vi "NR set HO Band.vi"(8 "error in (no error)":errorcluster caption="에러 입력(에러 없음)", 10 "Operation Band":u32, 11 "Instrument Manager 입력":refnum<class "Instrument Manager.lvclass">) -> (0 "error out":errorcluster caption="에러 출력", 3 "Instrument Manager 출력":refnum<class "Instrument Manager.lvclass">)   [LabVIEW 2023, in "Instrument Manager.lvclass"]
uses:
  Instrument Manager.lvclass
  Module/ANRITSU Call Box/Type Definition/NR Selected CC Type Arguments.ctl
  Instrument Manager.lvclass/Instrument Manager.ctl
  Module/ANRITSU Call Box/Interface Class/Anritsu Call Box.lvclass
  Module/ANRITSU Call Box/ANRITSU Call Box.lvlib
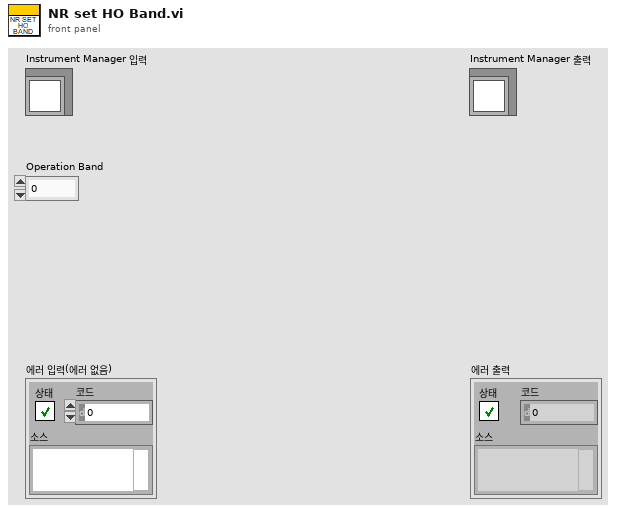
[diagram p1: front panel]
types:
  T1 = typedef "ANRITSU Call Box.lvlib/NR Selected CC Type Arguments.ctl" = cluster{"Selected CC":enum16{"PCC", "SCC", "FR2_PCC", "FR2_SCC"}, "SCC or FR2_SCC Index":u32}
  T2 = cluster{"Anritsu Call Box":refnum<class "Anritsu Call Box.lvclass">, "Spectrum Analyzer":refnum<class "Interface_Spectrum.lvclass">, "RF Switch Box":refnum<class "RF Filter Box.lvclass">, "Turn Table":refnum<class "Interface - Turn Table.lvclass">, "Mast":refnum<class "Interface - Mast.lvclass">, "3D Controller":refnum<class "Interface_3D Controller.lvclass">}
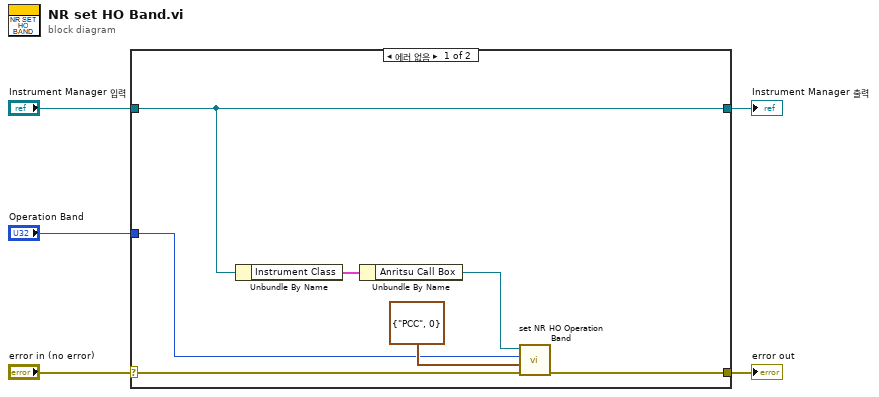
[diagram p0: block diagram]
diagram:
  n1 = case shown="에러 없음" "error in (no error)" {
    selector: "error in (no error)" -> [w11 w14]
    tunnel: [w10 w14] -> w4
    tunnel: [w8 w13] -> w2
    tunnel: "Instrument Manager 입력" -> [w8 w13]
    tunnel: "Operation Band" -> [w9 _]
    frame No Error {
      n2 = Unbundle By Name(w8) -> ("Instrument Class"=w7:T2)
      n3 = Unbundle By Name(w7) -> ("Anritsu Call Box"=w6:refnum<class "Anritsu Call Box.lvclass">)
      n4 = call-dynamic "set NR HO Operation Band.vi"("error in (no error)"=w11, "Selected CC Argements"=T1 {"Selected CC"=enum."PCC", "SCC or FR2_SCC Index"=0}, "Operation Band"=w9, "Anritsu Call Box 입력"=w6) -> ("error out"=w10:errorcluster)  [unwired: 6 in, 1 out]
    }
    frame Error {
    }
  }
  "error out" <- w4
  "Instrument Manager 출력" <- w2
